vi "Get Arduino Item(SubVI).vi"(10 "Item":string="X", 11 "String":string) -> (3 "Value":dbl)   [LabVIEW 2013]
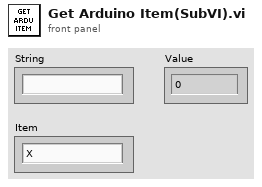
[diagram p1: front panel]
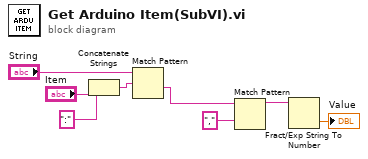
[diagram p0: block diagram]
diagram:
  n1 = Concatenate Strings("Item", ":" ("string")) -> (w3:string)
  n2 = Match Pattern(string="String", regular expression=w3) -> (after substring=w5:string)  [unwired: 1 in, 3 out]
  n3 = Match Pattern(string=w5, regular expression=",") -> (before substring=w7:string)  [unwired: 1 in, 3 out]
  n4 = Fract/Exp String To Number(string=w7) -> (number=→"Value":dbl)  [unwired: 3 in, 1 out]
